vi "Write_data_to_file.vi"(0 "start_path":path=path "C:/Users/IITH/Desktop/RK/Lab_view_automation/test_solenoid_SSR", 1 "Start_delay_ms":dbl=150.0, 2 "shot_data":dbl[][](array[numeric]), 3 "error_in":errorcluster, 4 "Actual_AI_Rate":dbl=300300.0) -> (5 "Write_OK":bool, 6 "file_path":path, 7 "error_out":errorcluster)   [LabVIEW 2025]
uses:
  <vilib>/Utility/file.llb/Write Delimited Spreadsheet (DBL).vi
panel:
  out "transposed_array":dbl[][](array[numeric]) format="%.4f"
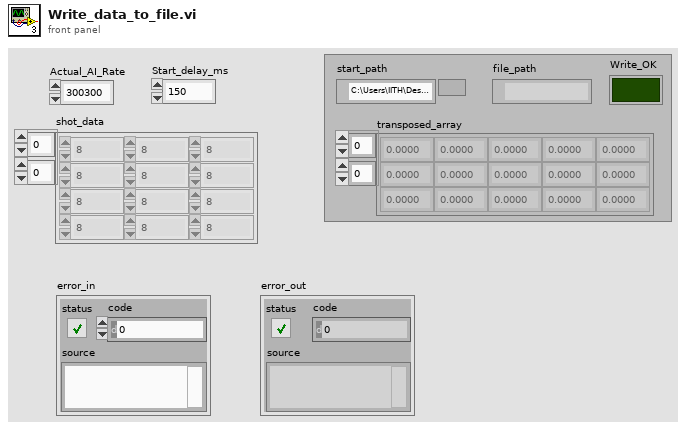
[diagram p1: front panel]
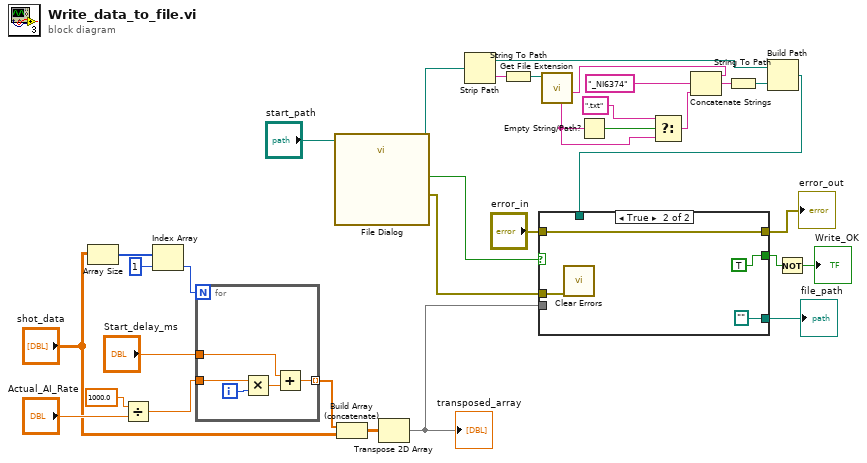
[diagram p0: block diagram]
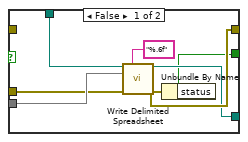
[diagram p2: hidden frame]
diagram:
  n1 = Array Size(array="shot_data") -> (size(s)=w31:i32[])
  n2 = Divide(x=1000.0, y="Actual_AI_Rate") -> (x/y=w26:dbl)
  n3 = Index Array(array=w31, index=1) -> (element=w30:i32)
  n4 = for {
    N: w30 -> [_]
    tunnel: [w35] -> w29 mode=indexing
    tunnel: w26 -> [w34]
    tunnel: "Start_delay_ms" -> [w33]
    i -> [w37]
    n5 = Multiply(x=w34, y=w37) -> (x*y=w36:dbl)
    n6 = Add(x=w33, y=w36) -> (x+y=w35:dbl)
  }
  n7 = call "File Dialog"("start path"="start_path") -> ("selected path"=w20:path, "cancelled"=w10:bool, "error out"=w1:errorcluster)  [unwired: 11 in, 1 out]
  n8 = Build Array (concatenate)(w29, "shot_data") -> (w28:dbl[][])
  n9 = Transpose 2D Array(2D array=w28) -> (transposed array=w6:dbl[][])
  "transposed_array" <- w6
  n10 = Strip Path(path=w20) -> (stripped path=w11:path, name=w19:string)
  n11 = String To Path(string=w19) -> (path=w18:path)
  n12 = call <vilib>:"Get File Extension.vi"("file"=w18) -> ("filename without extension"=w2:string, "unmodified file extension"=w15:string)  [unwired: 6 in, 3 out]
  n13 = Empty String/Path?(string/path=w15) -> (empty?=w17:bool)
  n14 = Select(t=".txt", s=w17, f=w15) -> (s? t:f=w14:string)
  n15 = Concatenate Strings(w2, "_NI6374" ("string"), w14) -> (w13:string)
  n16 = String To Path(string=w13) -> (path=w12:path)
  n17 = Build Path(base path=w11, name or relative path=w12) -> (appended path=w5:path)
  n18 = case shown="True" w10 {
    tunnel: [w39 TRUE] -> w3
    tunnel: "error_in" -> [_ w47]
    tunnel: [w42 w47] -> w8
    tunnel: [w41 path ""] -> w7
    tunnel: w6 -> [w44 _]
    tunnel: w5 -> [w40 _]
    tunnel: w1 -> [w38 w45]
    frame False {
      n19 = call-poly <vilib>:"Write Delimited Spreadsheet.vi"("file path (dialog if empty)"=w40, "format (%.3f)"="%.6f", "2D data"=w44, "error in (no error)"=w38) -> ("new file path (Not A Path if cancelled)"=w41:path, "error out"=w42:errorcluster)  [unwired: 10 in]
      n20 = Unbundle By Name(w42) -> ("status"=w39:bool)
    }
    frame True {
      n21 = call <vilib>:"Clear Errors.vi"("error in (no error)"=w45) -> ()  [unwired: 5 in, 2 out]
    }
  }
  "file_path" <- w7
  "error_out" <- w8
  n22 = Not(x=w3) -> (.not. x?=→"Write_OK":bool)
